vi "Check SPI Device.vi"(8 "error in (no error)":errorcluster, 11 "SPI Device":T1) -> (0 "error out":errorcluster, 3 "SPI Device out":T1)   [LabVIEW 2020, in "wiringPi.lvlib"]
doc: "<b>_______________________________________________________________</b>\n** Author: Juan José Villacorta\n** LabVIEW wrapper for C library <b> wiringPi </b>,\n** https://github.com/WiringPi/WiringPi\n<b>_______________________________________________________________</b>\n/*\n * Check if the SPI device is present\n**********************************************************************************\n*/"
uses:
  wiringPi.lvlib
  <vilib>/ErrorRing/Error Ring.xnode
  <vilib>/Utility/error.llb/Error Cluster From Error Code.vi
  Type Defs/SPI Dev.ctl
  Type Defs/SPI Channel.ctl
  Type Defs/SPI Device.ctl
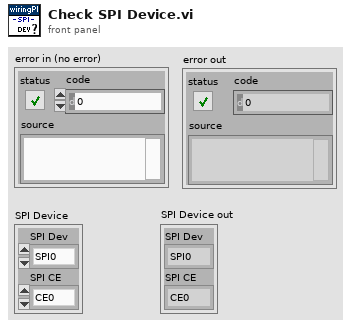
[diagram p1: front panel]
types:
  T1 = typedef "wiringPi.lvlib/SPI Device.ctl" = cluster{"SPI Dev":T2, "SPI CE":T3}
  T2 = typedef "wiringPi.lvlib/SPI Dev.ctl" = enum32{"SPI0", "SPI1"}
  T3 = typedef "wiringPi.lvlib/SPI Channel.ctl" = enum32{"CE0", "CE1", "CE2"}
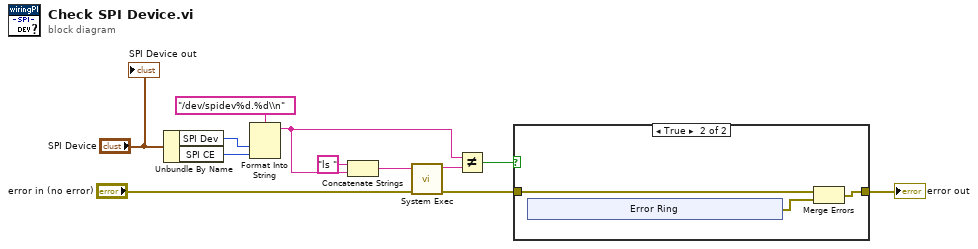
[diagram p0: block diagram]
diagram:
  n1 = Unbundle By Name("SPI Device") -> ("SPI Dev"=w10:T2, "SPI CE"=w11:T3)
  n2 = Format Into String(format string="/dev/spidev%d.%d\\n", w10, w11) -> (resulting string=w4:string)  [unwired: 2 in, 1 out]
  n3 = Concatenate Strings("ls " ("string"), w4) -> (w7:string)
  n4 = call <vilib>:"System Exec.vi"("error in (no error)"="error in (no error)", "command line"=w7) -> ("error out"=w2:errorcluster, "standard output"=w5:string)  [unwired: 6 in, 2 out]
  n5 = Not Equal?(x=w4, y=w5) -> (x != y?=w3:bool)
  n6 = case shown="True" w3 {
    tunnel: w2 -> [w13 w15]
    tunnel: [w13 w14] -> w1
    frame False {
    }
    frame True {
      n7 = xnode "Error Ring"() -> ("error out"=w16:errorcluster)
      n8 = Merge Errors(w15, w16) -> (w14:errorcluster)
    }
  }
  "error out" <- w1
  "SPI Device out" <- "SPI Device"
